vi "delayMicroseconds.vi"(8 "error in (no error)":errorcluster, 11 "us":u32=1000) -> (0 "error out":errorcluster)   [LabVIEW 2025, in "wiringPi.lvlib"]
doc: "<b>_______________________________________________________________</b>\n** Author: Juan José Villacorta\n** LabVIEW wrapper for C library <b> wiringPi </b>,\n** https://github.com/WiringPi/WiringPi\n<b>_______________________________________________________________</b>\n\n/*\n * delayMicroseconds:\n * This is somewhat intersting. It seems that on the Pi, a single call\n * to nanosleep takes some 80 to 130 microseconds anyway, so while\n * obeying the standards (may take longer), it's not always what we\n * want!\n *\n * So what I'll do now is if the delay is less than 100uS we'll do it\n * in a hard loop, watching a built-in counter on the ARM chip. This is\n * somewhat sub-optimal in that it uses 100% CPU, something not an issue\n * in a microcontroller, but under a multi-tasking, multi-user OS, it's\n * wastefull, however we've no real choice )-:\n *\n * Plan B: It seems all might not be well with that plan, so changing it\n * to use gettimeofday () and poll on that instead...\n *********************************************************************************\n */"
uses:
  wiringPi.lvlib
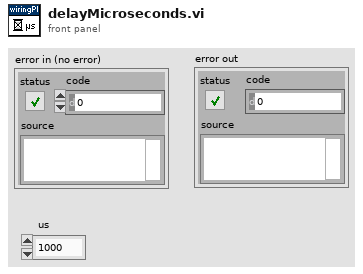
[diagram p1: front panel]
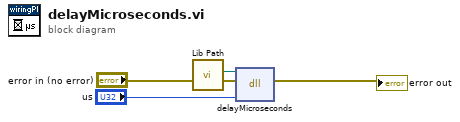
[diagram p0: block diagram]
diagram:
  n1 = call "Lib Path.vi"() -> ("path out"=w1:path)  [unwired: 11 in]
  n2 = dll-call lib="libLVwiringPI.so" fn="delayMicroseconds"(path in=w1, error in="error in (no error)", "ms"="us") -> (error out=→"error out":errorcluster)  [unwired: 3 in, 1 out]
